vi "niSwitch Attach gRPC Session.vi"(5 "gRPC options":T1={"session name"="", "address (localhost)"="localhost", "port (31763)"=31763}, 8 "error in":errorcluster) -> (0 "error out":errorcluster, 3 "session factory out":refnum<class "Session Factory.lvclass">)   [LabVIEW 2021, in "Session Management niSwitch.lvlib" / "Session Factory.lvclass"]
doc: "Attaches to an existing NI-Switch session with the specified <b>session name</b> on the specified NI gRPC Device Server. Returns a session factory object to be used in all subsequent NI-Switch calls.\n\n<B>NOTE:</B> If you do not specify a session name for the server, or if the specified session name did not previously exist on the server, then NI-Switch will return an error."
uses:
  Session Factory.lvclass
  niSwitch gRPC Device Server.ctl
  NI Switch Client/RPC Messages/niswitch_grpc_InitWithTopologyRequest.ctl
  NI Switch Client/RPC Messages/nidevice_grpc_SessionInitializationBehavior.ctl
  Session Factory.lvclass/Session Factory.ctl
  NI Switch Client/NI Switch Client.lvlib
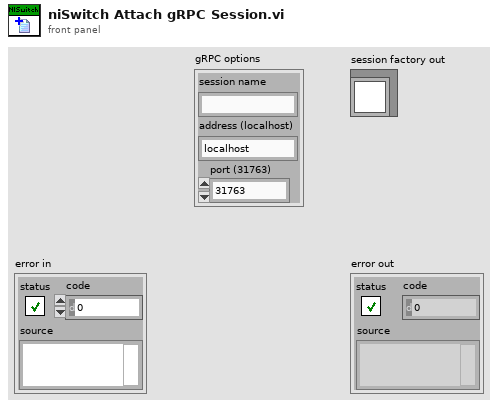
[diagram p1: front panel]
types:
  T1 = typedef "Session Management niSwitch.lvlib/Session Factory.lvclass/niSwitch gRPC Device Server.ctl" = cluster{"session name":string, "address (localhost)":string, "port (31763)":u32}
  T2 = typedef "NI Switch Client.lvlib/nidevice_grpc_SessionInitializationBehavior.ctl" = enum32{"SESSION_INITIALIZATION_BEHAVIOR_UNSPECIFIED", "SESSION_INITIALIZATION_BEHAVIOR_INITIALIZE_NEW", "SESSION_INITIALIZATION_BEHAVIOR_ATTACH_TO_EXISTING"}
  T3 = typedef "NI Switch Client.lvlib/niswitch_grpc_InitWithTopologyRequest.ctl" = cluster{"session_name":string, "resource_name":string, "topology":string, "simulate":bool, "reset_device":bool, "initialization_behavior":T2}
  T4 = typedef "grpc-lvsupport-release.lvlib/grpcId.ctl" = u64
  T5 = typedef "NI Switch Client.lvlib/niswitch_grpc_InitWithTopologyResponse.ctl" = cluster{"status":i32, "vi":T6, "error_message":string, "new_session_initialized":bool}
  T6 = typedef "NI Switch Client.lvlib/nidevice_grpc_Session.ctl" = cluster{"nidevice_grpc_Session_session":refnum<class "nidevice_grpc_Session_session.lvclass">}
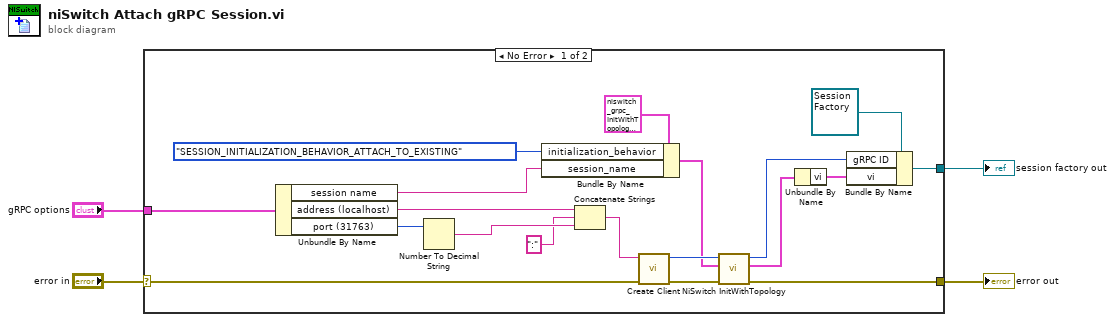
[diagram p0: block diagram]
diagram:
  n1 = case shown="No Error" "error in" {
    selector: "error in" -> [w15 w24]
    tunnel: [w8 w24] -> w1
    tunnel: [w18 _] -> w4
    tunnel: "gRPC options" -> [w16 _]
    frame No Error {
      n2 = Unbundle By Name(w16) -> ("session name"=w11:string, "address (localhost)"=w13:string, "port (31763)"=w14:u32)
      n3 = Number To Decimal String(number=w14) -> (decimal integer string=w12:string)  [unwired: 1 in]
      n4 = Bundle By Name(cluster=T3 {"session_name"="", "resource_name"="", "topology"="", "simulate"=FALSE, "reset_device"=FALSE, "initialization_behavior"=enum."SESSION_INITIALIZATION_BEHAVIOR_UNSPECIFIED"} ("Request Data"), "initialization_behavior"=nidevice_grpc_SessionInitializationBehavior."SESSION_INITIALIZATION_BEHAVIOR_ATTACH_TO_EXISTING", "session_name"=w11) -> (w17:T3)
      n5 = Concatenate Strings(w13, ":" ("string"), w12) -> (w5:string)
      n6 = call "Create Client.vi"("error in"=w15, "address"=w5) -> ("error out"=w9:errorcluster, "gRPC ID Out"=w23:T4)  [unwired: 8 in]
      n7 = call "NiSwitch InitWithTopology.vi"("error in"=w9, "Request Data"=w17, "gRPC ID"=w23) -> ("error out"=w8:errorcluster, "Response Data"=w20:T5, "gRPC ID out"=w22:T4)  [unwired: 6 in]
      n8 = Unbundle By Name(w20) -> ("vi"=w21:T6)
      n9 = Bundle By Name(cluster=refnum<class "Session Factory.lvclass"> refnum ("NI Session Management niSwitch.lvlib:Session Factory.lvclass"), "gRPC ID"=w22, "vi"=w21) -> (w18:refnum<class "Session Factory.lvclass">)
    }
    frame Error {
    }
  }
  "error out" <- w1
  "session factory out" <- w4
